vi "FOV_Zoom_Frame to Hex.vi"(5 "timings_offsets":dbl[](array[numeric]), 7 "distortion_corr":dbl, 8 "Objective":i8=20, 9 "Z pixel Size":i8=4, 11 "AOL_Globals":T1={"Imaging Protocol"=enum."AOL Z-Stack", "Number of POI"=0, "Number of Miniscans"=0, "Number of Trials"=0, "Number of Cycles "=0, "# Averaged Frames"=0, "Laser power (%)"=0, "Pockels (V)"=0.0, "Acquisition Length (sec)"=0.0, "Fill time (us)"=0.0, "POI Dwell time (us)"=0.0, "Miniscan Dwell time per pixel (us)"=0.0, "PMT 1"=0.0, "PMT 2"=0.0, "Back Apperture (mA)"=0.0, "Frame Size"=0, "Center Frequency"=0.0, "Field of View (um)"=175.0, "Field of View (norm)"=0.0, "DwellTime (us)"=0.0, "Ref Dwell Time (us)"=0.0, "Wavelength (nm)"=0.0, "Zoom"=0.0, "AOL Z"=0.0, "AOL Mode"=enum."Raster", "GridXY"=0.0, "GridZ"=0.0, "TriggerPeriod (sec)"=0.0, "Number of Pixels in Miniscan"=0, "Experiment folder path"=path "", "X centre"=0.0, "Y centre"=0.0, "Angle (degrees)"=0.0, "Angle Xs (degrees)"=0.0, "Angle Ys (degrees)"=0.0, "Plane Mode"=0, "Threshold"=[], "Regenerate Chirps"=FALSE, "Rectangle ROI length (pixels)"=0, "Rectangle ROI height (pixels)"=0, "AOD fill"=4900, "StartupDelay"=0, "Samples Wait after Trigger"=5080, "Slip Cycle"=600000, "Add Cycle"=TRUE, "Functional Mode"=enum."Point", "Z Start"=0.0, "Z Stop"=0.0, "# Planes"=0, "Total Pixels"=0, "Variable Miniscan Pixels"=[], "Use Variable Length"=FALSE, "Use Variable Resolution"=FALSE, "Laser power (%) at Z Start"=0, "Laser power (%) at Z Stop"=0, "Ref Z Step"=0} {"Angle Ys (degrees)" format="%#.6g"; "Angle Xs (degrees)" format="%#.6g"; "Plane Mode" items=["XY Plane", "XZ Plane", "YZ Plane", "arbitraryplane"]; "Frame Size" items=["100X100"=100, "128X128"=128, "200X200"=200, "256X256"=256, "512X512"=512, "1024x1024"=1024, "2048x2048"=2048]; "Back Apperture (mA)" format="%#.6g"; "Pockels (V)" format="%#.6g"; "PMT 2" format="%#.6g"; "PMT 1" format="%#.6g"; "Angle (degrees)" format="%#.6g"; "POI Dwell time (us)" format="%#.6g"}) -> (3 "FOV-Zoom-FrameSize Hex":string)   [LabVIEW 2020]
uses:
  Typedefs/Controls/AOL_Globals.ctl
  Typedefs/Imaging Protocols enum.ctl
  Typedefs/Frame Size.ctl
  Typedefs/AOL modes.ctl
  Typedefs/Plane Mode.ctl
  Typedefs/Functional Mode.ctl
  <vilib>/Utility/miscctls.llb/LVStringsAndValuesArrayTypeDef_SGL.ctl
panel:
  out "length":i32
  out "Field of view (um)":dbl
  # "SUBROUTINE"
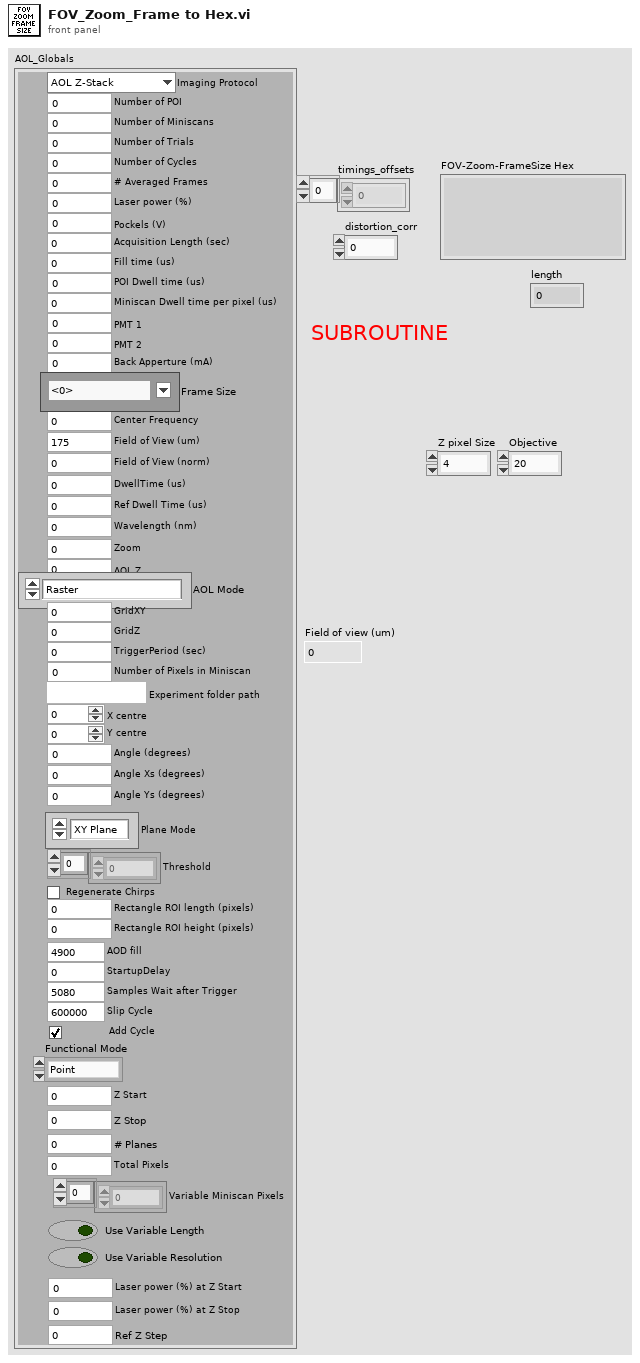
[diagram p1: front panel]
types:
  T1 = typedef "AOL_Globals.ctl" = cluster{"Imaging Protocol":T2, "Number of POI":u16, "Number of Miniscans":u16, "Number of Trials":u16, "Number of Cycles ":u64, "# Averaged Frames":u16, "Laser power (%)":u8, "Pockels (V)":dbl, "Acquisition Length (sec)":dbl, "Fill time (us)":dbl, "POI Dwell time (us)":dbl, "Miniscan Dwell time per pixel (us)":dbl, "PMT 1":dbl, "PMT 2":dbl, "Back Apperture (mA)":dbl, "Frame Size":T3, "Center Frequency":dbl, "Field of View (um)":dbl, "Field of View (norm)":dbl, "DwellTime (us)":dbl, "Ref Dwell Time (us)":dbl, "Wavelength (nm)":dbl, "Zoom":dbl, "AOL Z":dbl, "AOL Mode":T4, "GridXY":dbl, "GridZ":dbl, "TriggerPeriod (sec)":dbl, "Number of Pixels in Miniscan":u16, "Experiment folder path":path, "X centre":dbl, "Y centre":dbl, "Angle (degrees)":dbl, "Angle Xs (degrees)":dbl, "Angle Ys (degrees)":dbl, "Plane Mode":T5, "Threshold":u16[], "Regenerate Chirps":bool, "Rectangle ROI length (pixels)":u16, "Rectangle ROI height (pixels)":u16, "AOD fill":u16, "StartupDelay":i32, "Samples Wait after Trigger":u16, "Slip Cycle":u32, "Add Cycle":bool, "Functional Mode":T6, "Z Start":dbl, "Z Stop":dbl, "# Planes":i32, "Total Pixels":i32, "Variable Miniscan Pixels":u16[], "Use Variable Length":bool, "Use Variable Resolution":bool, "Laser power (%) at Z Start":u8, "Laser power (%) at Z Stop":u8, "Ref Z Step":i8}
  T2 = typedef "Imaging Protocols enum.ctl" = enum16{"AOL Z-Stack", "Motor Z Stack", "Parameter Sweep", "Functional Acquisition", "Single Plane Acquisition", "Volume Acquisition", "Live Imaging", "Live Plane Imaging", "Live Volume Imaging"}
  T3 = typedef "Frame Size.ctl" = u16
  T4 = typedef "AOL modes.ctl" = enum16{"Raster", "Structural", "Pointing", "Mini Scan", "Alignment"}
  T5 = typedef "Plane Mode.ctl" = u16
  T6 = typedef "Functional Mode.ctl" = enum16{"Point", "Line", "Patch", "Plane", "Volume"}
  T7 = typedef "LVStringsAndValuesArrayTypeDef_SGL.ctl" = cluster{"String":string, "Value":sgl}[]
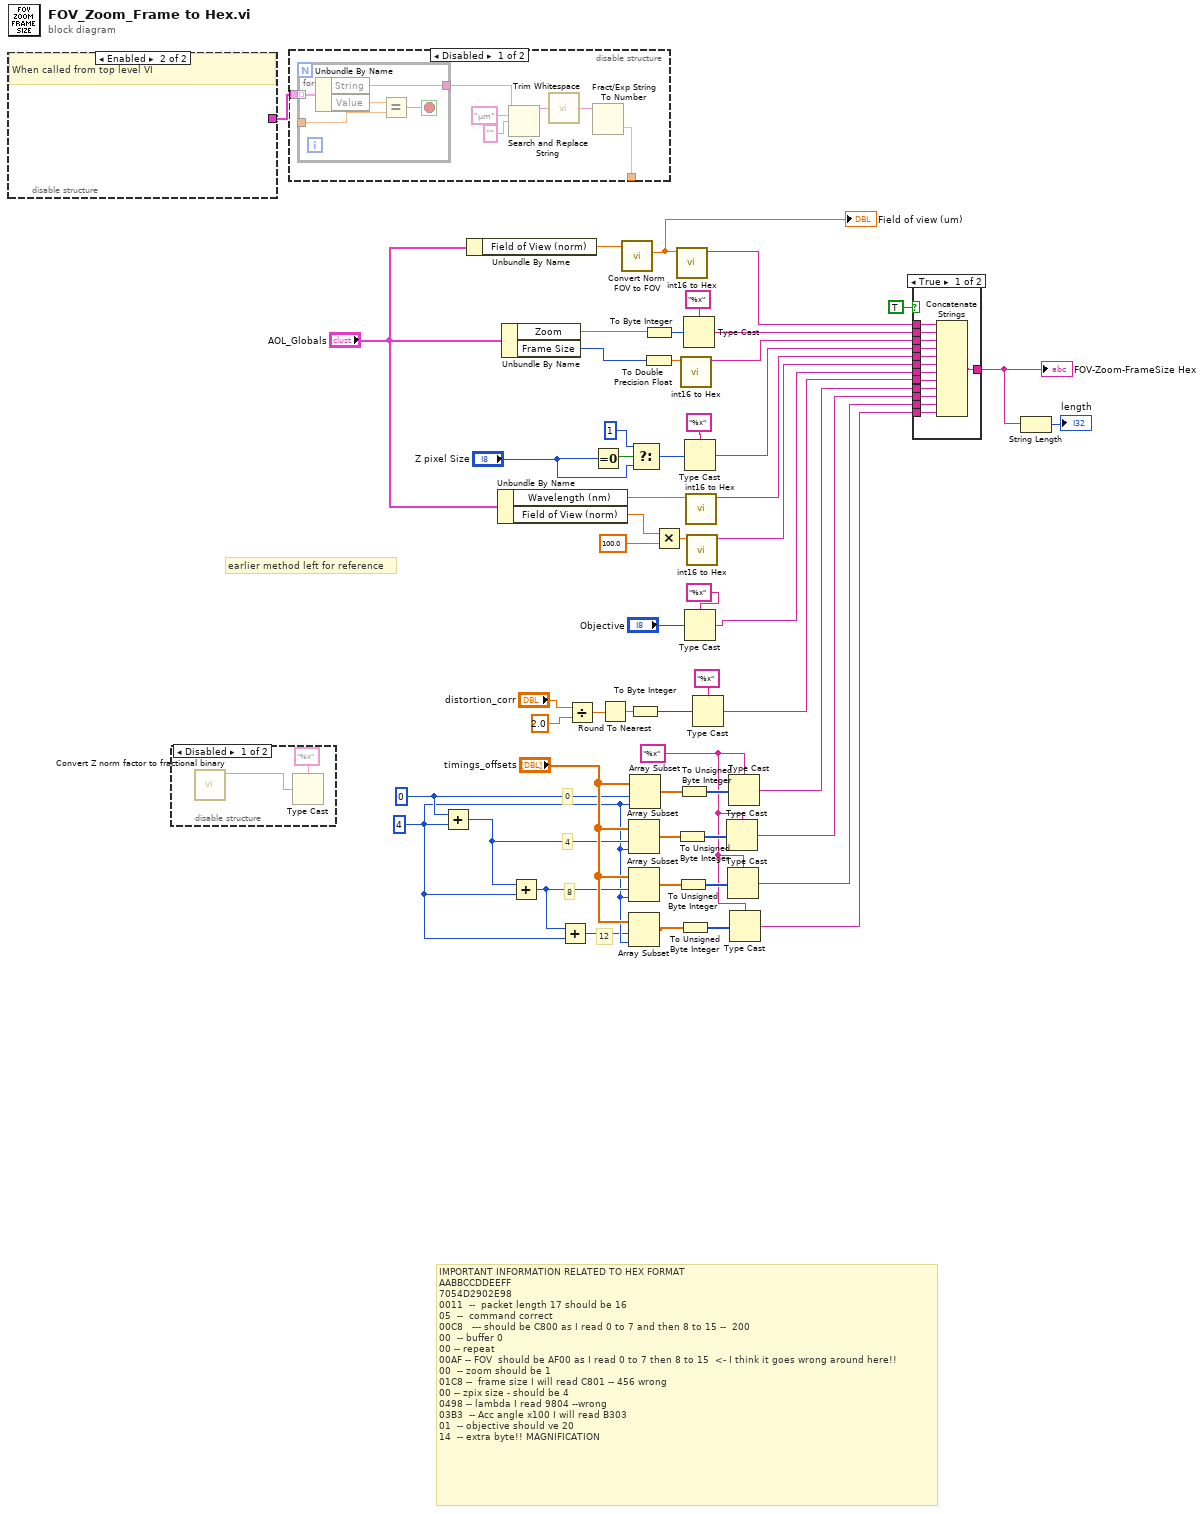
[diagram p0: block diagram]
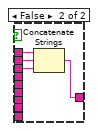
[diagram p4: hidden frame]
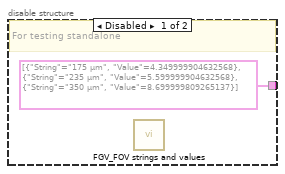
[diagram p5: hidden frame]
diagram:
  w9 = 4 ("y")
  w12 = 0 ("index")
  w17 = "%x" ("type")
  # "earlier method left for reference"
  # "12"
  # "8"
  # "4"
  # "0"
  # "IMPORTANT INFORMATION RELATED TO HEX FORMAT\nAABBCCDDEEFF\n7054D2902E98\n0011  --  packet length 17 should be 16\n05  --  command correct\n00C8   --- should be C800 as I read 0 to 7 and then 8 to 15 --  200\n00  -- buffer 0\n00 -- repeat\n00AF -- FOV  should be AF00 as I read 0 to 7 then 8 to 15  <- I think it goes wrong around here!!\n00  -- zoom should be 1\n01C8 --  frame size I will read C801 -- 456 wrong\n00 -- zpix size - should be 4\n0498 -- lambda I read 9804 --wrong\n03B3  -- Acc angle x100 I will read B303\n01  -- objective should ve 20\n14  -- extra byte!! MAGNIFICATION"
  n1 = disable-structure shown="Enabled" {
    disable-tunnel: [T7 [{"String"="175 µm", "Value"=4.35}, {"String"="235 µm", "Value"=5.6}, {"String"="350 µm", "Value"=8.7}] ("Strings And Values []") _] -> w48
    frame Disabled {
      # "For testing standalone"
      n2 = call "FGV_FOV strings and values.vi"() -> ()  [unwired: 10 in, 2 out]
    }
    frame Enabled {
      # "When called from top level VI"
    }
  }
  n3 = disable-structure shown="Disabled" {
    frame Disabled {
      n4 = call "Convert Z norm factor to fractional binary.vi"() -> ("Fractional Z norm factor"=w58:u8)  [unwired: 11 in]
      n5 = Type Cast(type="%x", x=w58) -> ()  [unwired: 1 out]
    }
    frame Enabled {
    }
  }
  n6 = disable-structure shown="Disabled" {
    disable-tunnel: [w61 _] -> _
    disable-tunnel: w48 -> [w60 _]
    frame Disabled {
      n7 = for {
        tunnel: _ -> [w69]
        tunnel: w60 -> [w71] mode=indexing
        tunnel: [w67] -> w62
        stop <- w68 stop-if-true
        n8 = Unbundle By Name(w71) -> ("String"=w67:string, "Value"=w70:sgl)
        n9 = Equal?(x=w70, y=w69) -> (x = y?=w68:bool)
      }
      n10 = Search and Replace String(input string=w62, search string="µm", replace string="" ("replace string (\"\")")) -> (result string=w65:string)  [unwired: 5 in, 3 out]
      n11 = call <vilib>:"Trim Whitespace.vi"("string"=w65) -> ("trimmed string"=w66:string)  [unwired: 1 in]
      n12 = Fract/Exp String To Number(string=w66) -> (number=w61:dbl)  [unwired: 3 in, 1 out]
    }
    frame Enabled {
    }
  }
  n13 = Add(x=w12, y=w9) -> (x+y=w11:i32)
  n14 = Unbundle By Name("AOL_Globals") -> ("Field of View (norm)"=w34:dbl)
  n15 = Unbundle By Name("AOL_Globals") -> ("Wavelength (nm)"=w47:dbl, "Field of View (norm)"=w45:dbl)
  n16 = Unbundle By Name("AOL_Globals") -> ("Zoom"=w52:dbl, "Frame Size"=w56:T3)
  n17 = Add(x=w11, y=w9) -> (x+y=w10:i32)
  n18 = Add(x=w10, y=w9) -> (x+y=w8:i32)
  n19 = Divide(x="distortion_corr", y=2.0) -> (x/y=w5:dbl)
  n20 = Equal To 0?(x="Z pixel Size") -> (x = 0?=w36:bool)
  n21 = Round To Nearest(number=w5) -> (nearest integer value=w4:dbl)
  n22 = call "Convert Norm FOV to FOV.vi"("Field of View(norm)"=w34) -> ("FOV"=w33:dbl)  [unwired: 9 in, 1 out]
  "Field of view (um)" <- w33
  n23 = Array Subset(array="timings_offsets", index=w11, length=w9) -> (w22:dbl[])
  n24 = Array Subset(array="timings_offsets", index=w10, length=w9) -> (w18:dbl[])
  n25 = Array Subset(array="timings_offsets", index=w8, length=w9) -> (w19:dbl[])
  n26 = To Byte Integer(number=w4) -> (8bit integer=w27:i8)
  n27 = Array Subset(array="timings_offsets", index=w12, length=w9) -> (w25:dbl[])
  n28 = Select(t=i8 1, s=w36, f="Z pixel Size") -> (s? t:f=w37:i8)
  n29 = To Byte Integer(number=w52) -> (8bit integer=w53:i8)
  n30 = To Double Precision Float(number=w56) -> (double precision float=w55:dbl)
  n31 = Multiply(x=w45, y=100.0) -> (x*y=w46:dbl)
  n32 = call "int16 to Hex.vi"("number"=w33) -> ("Hex string"=w51:string)  [unwired: 10 in]
  n33 = To Unsigned Byte Integer(number=w22) -> (unsigned 8bit integer=w23:u8[])
  n34 = To Unsigned Byte Integer(number=w18) -> (unsigned 8bit integer=w21:u8[])
  n35 = To Unsigned Byte Integer(number=w25) -> (unsigned 8bit integer=w24:u8[])
  n36 = To Unsigned Byte Integer(number=w19) -> (unsigned 8bit integer=w20:u8[])
  n37 = call "int16 to Hex.vi"("number"=w55) -> ("Hex string"=w49:string)  [unwired: 10 in]
  n38 = Type Cast(type="%x", x=w53) -> (*(type *) &x=w50:string)
  n39 = Type Cast(type="%x", x=w37) -> (*(type *) &x=w42:string)
  n40 = Type Cast(type="%x", x="Objective") -> (*(type *) &x=w1:string)
  n41 = call "int16 to Hex.vi"("number"=w47) -> ("Hex string"=w41:string)  [unwired: 10 in]
  n42 = call "int16 to Hex.vi"("number"=w46) -> ("Hex string"=w32:string)  [unwired: 10 in]
  n43 = Type Cast(type="%x", x=w27) -> (*(type *) &x=w28:string)
  n44 = Type Cast(type=w17, x=w23) -> (*(type *) &x=w15:string)
  n45 = Type Cast(type=w17, x=w21) -> (*(type *) &x=w14:string)
  n46 = Type Cast(type=w17, x=w24) -> (*(type *) &x=w16:string)
  n47 = Type Cast(type=w17, x=w20) -> (*(type *) &x=w13:string)
  n48 = case shown="True" TRUE {
    tunnel: w51 -> [w84 w88]
    tunnel: w50 -> [w83 w87]
    tunnel: w49 -> [w82 w86]
    tunnel: [w81 w85] -> w29
    tunnel: w42 -> [w80 _]
    tunnel: w41 -> [w79 _]
    tunnel: w32 -> [w78 _]
    tunnel: w1 -> [w77 _]
    tunnel: w28 -> [w76 _]
    tunnel: w16 -> [w75 _]
    tunnel: w15 -> [w74 _]
    tunnel: w14 -> [w73 _]
    tunnel: w13 -> [w72 _]
    frame True {
      n49 = Concatenate Strings(w84, w83, w82, w80, w79, w78, w77, w76, w75, w74, w73, w72) -> (w81:string)
    }
    frame False {
      n50 = Concatenate Strings(w88, w87, w86) -> (w85:string)
    }
  }
  "FOV-Zoom-FrameSize Hex" <- w29
  n51 = String Length(string=w29) -> (length=→"length":i32)
